vi "Configure Module.vi"(8 "error in (no error)":errorcluster, 10 "IOV ref in":variant, 11 "9403 in":refnum<class "9403.lvclass">) -> (0 "error out":errorcluster, 2 "IOV ref out":variant, 3 "9403 out":refnum<class "9403.lvclass">)   [LabVIEW 2020, in "Modules.lvlib" / "9403.lvclass"]
uses:
  9403.lvclass
  <resource>/objmgr/cRIO.rc
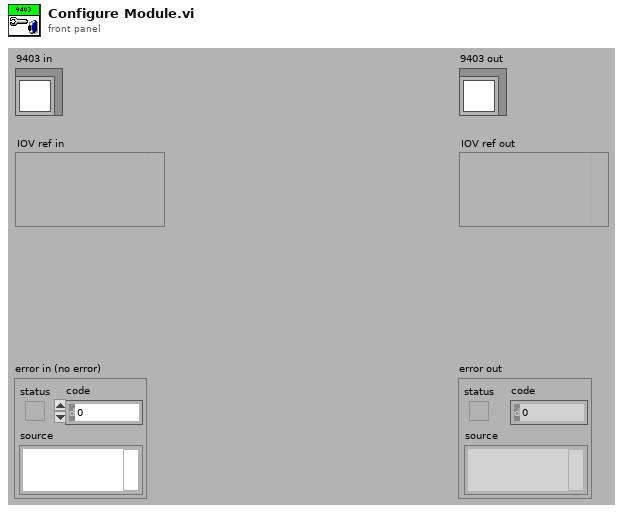
[diagram p1: front panel]
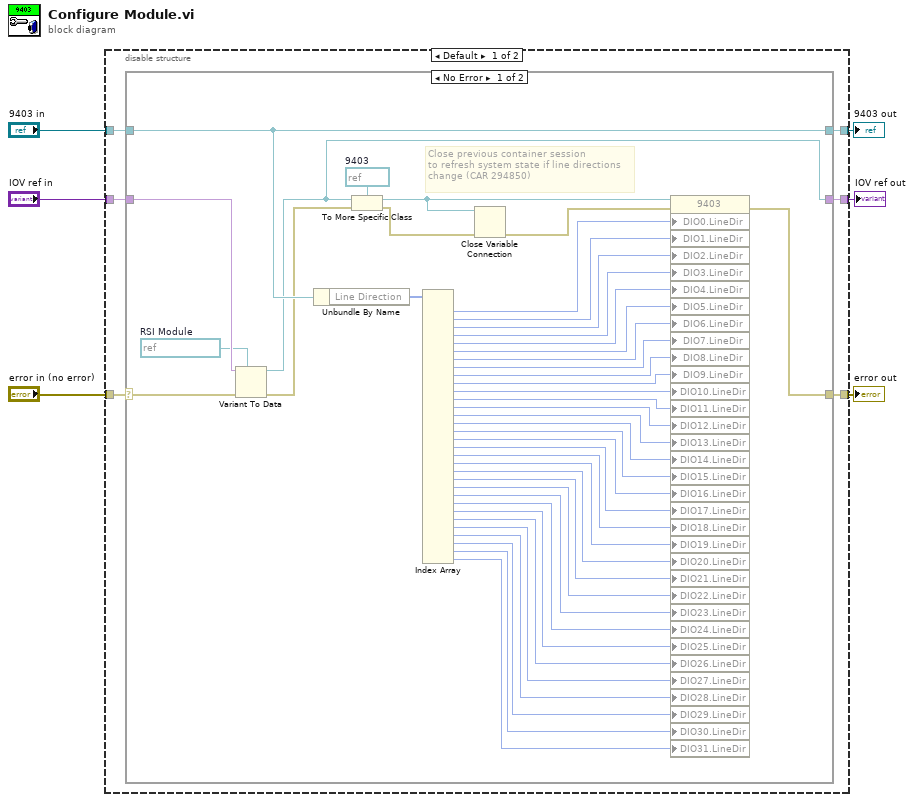
[diagram p0: block diagram]
diagram:
  n1 = disable-structure shown="Default" {
    disable-tunnel: "error in (no error)" -> [w12 w62]
    disable-tunnel: [w11 w62] -> w5
    disable-tunnel: "9403 in" -> [w10 w60]
    disable-tunnel: [w9 w60] -> w3
    disable-tunnel: "IOV ref in" -> [w8 w61]
    disable-tunnel: [w7 w61] -> w1
    frame condition #0 {
      n2 = case shown="No Error" w12 {
        selector: w12 -> [w55 w59]
        tunnel: [w53 w59] -> w11
        tunnel: [w56 w58] -> w9
        tunnel: w10 -> [w56 w58]
        tunnel: w8 -> [w15 w57]
        tunnel: [w14 w57] -> w7
        frame No Error {
          w13 = refnum<k21> refnum  # RSI Module
          w54 = refnum<k21> refnum  # 9403
          # "Close previous container session\nto refresh system state if line directions\nchange (CAR 294850)"
          n3 = Variant To Data(error in=w55, type=w13, Variant=w15) -> (data=w14:refnum<k21>, error out=w16:errorcluster)
          n4 = Unbundle By Name(w56) -> ("Line Direction"=w52:u32[])
          n5 = To More Specific Class(target class=w54, reference=w14, error in=w16) -> (specific class reference=w19:refnum<k21>, error out=w18:errorcluster)
          n6 = Index Array(array=w52) -> (element #1=w51:u32, element #2=w50:u32, element #3=w49:u32, element #4=w48:u32, element #5=w47:u32, element #6=w46:u32, element #7=w45:u32, element #8=w44:u32, element #9=w43:u32, element #10=w42:u32, element #11=w41:u32, element #12=w40:u32, element #13=w39:u32, element #14=w38:u32, element #15=w37:u32, element #16=w36:u32, element #17=w35:u32, element #18=w34:u32, element #19=w33:u32, element #20=w32:u32, element #21=w31:u32, element #22=w30:u32, element #23=w29:u32, element #24=w28:u32, element #25=w27:u32, element #26=w26:u32, element #27=w25:u32, element #28=w24:u32, element #29=w23:u32, element #30=w22:u32, element #31=w21:u32, element #32=w20:u32)  [unwired: 32 in]
          n7 = Close Variable Connection(8:w18, 11:w19) -> (0:w17:errorcluster)
          n8 = property class="9403"(reference=w19, error in=w17, "DIO0.LineDir"=w51, "DIO1.LineDir"=w50, "DIO2.LineDir"=w49, "DIO3.LineDir"=w48, "DIO4.LineDir"=w47, "DIO5.LineDir"=w46, "DIO6.LineDir"=w45, "DIO7.LineDir"=w44, "DIO8.LineDir"=w43, "DIO9.LineDir"=w42, "DIO10.LineDir"=w41, "DIO11.LineDir"=w40, "DIO12.LineDir"=w39, "DIO13.LineDir"=w38, "DIO14.LineDir"=w37, "DIO15.LineDir"=w36, "DIO16.LineDir"=w35, "DIO17.LineDir"=w34, "DIO18.LineDir"=w33, "DIO19.LineDir"=w32, "DIO20.LineDir"=w31, "DIO21.LineDir"=w30, "DIO22.LineDir"=w29, "DIO23.LineDir"=w28, "DIO24.LineDir"=w27, "DIO25.LineDir"=w26, "DIO26.LineDir"=w25, "DIO27.LineDir"=w24, "DIO28.LineDir"=w23, "DIO29.LineDir"=w22, "DIO30.LineDir"=w21, "DIO31.LineDir"=w20) -> (error out=w53:errorcluster)  [unwired: 1 out]
        }
        frame Error {
        }
      }
    }
    frame condition #1 (active) {
    }
  }
  "error out" <- w5
  "9403 out" <- w3
  "IOV ref out" <- w1
